vi "FuncVI-WaitUntil.vi"(5 "InstanceRef":T2, 9 "arg list":T1[](array[typedef]) {"num" format="%.2f"}) -> (0 "error out":bool, 3 "result":T1 {"num" format="%.2f"})   [LabVIEW 2021]
doc: "::: CalcExpress Toolkit :::\nCopyright (c) 2000-2026 Konstantin Shifershteyn. All rights reserved."
uses:
  cetypes.llb/CalcExpress Function Argument Info.ctl
  cetypes.llb/CalcExpress Instance RefNum.ctl
panel:
  in  "max arg num":i32=1
  in  "min arg num":i32
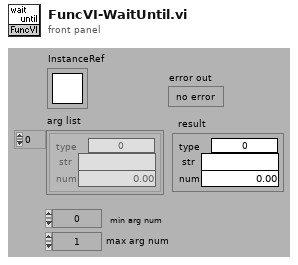
[diagram p1: front panel]
types:
  T1 = typedef "CalcExpress Function Argument Info.ctl" = cluster{"type":u32, "str":string, "num":dbl}
  T2 = typedef "CalcExpress Instance RefNum.ctl" = refnum<k1>
  T3 = enum8{"String", "DBL Number", "identifier", "1D Array of DBL", "2D Array of DBL", "CDB Number", "1D Array of CDB", "2D Array of CDB", "1D Array of String", "2D Array of String", "Unknown data type"}
  T4 = cluster{"type":enum8{"String", "DBL Number", "identifier", "1D Array of DBL", "2D Array of DBL", "CDB Number", "1D Array of CDB", "2D Array of CDB", "1D Array of String", "2D Array of String", "Unknown data type"}, string, "num val":dbl}
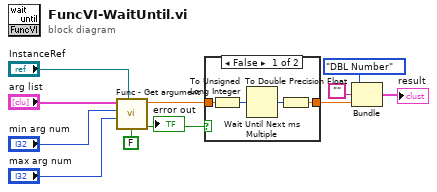
[diagram p0: block diagram]
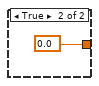
[diagram p2: hidden frame]
diagram:
  n1 = call "Func - Get argument.vi"("ena NonNum? (F)"=FALSE, "InstanceRef"="InstanceRef", "max arg num"="max arg num", "arg idx"="min arg num", "arg list"="arg list") -> ("error out"=w9:bool, "num"=w5:dbl)  [unwired: 1 in, 2 out]
  "error out" <- w9
  n2 = case shown="False" w9 {
    tunnel: w5 -> [w15 _]
    tunnel: [w12 0.0 ("num val")] -> w4
    frame False {
      n3 = To Unsigned Long Integer(number=w15) -> (unsigned 32bit integer=w14:u32)
      n4 = Wait Until Next ms Multiple(millisecond multiple=w14) -> (millisecond timer value=w13:u32)
      n5 = To Double Precision Float(number=w13) -> (double precision float=w12:dbl)
    }
    frame True {
    }
  }
  n6 = Bundle("type"=T3."DBL Number", "", "num val"=w4) -> (→"result":T4)  [unwired: 1 in]
